vi "PicoReadPicoStreamingBuffers.vi"(1 "enabled array":i16[](array[numeric]), 2 "Buffer and Transfer Settings":T2={"startIndex"=0, "Samples"=1000000, "Down Sample Ratio"=1, "Down-Sample Mode"=2147483648} {"Down-Sample Mode" items=["RAW none"=2147483648, "None"=0, "Aggregate"=1, "Decimate"=2, "Average"=4]; "Down Sample Ratio" step=1; "Samples" format="%_6p"}, 3 "Variant":string, 5 "Pointer array":u64[][](array[numeric]), 7 "Offset Index":u32, 9 "Number of Samples":u32, 11 "error in (no error)":errorcluster) -> (6 "Buffers (Max or non-aggregated)":T1, 8 "Buffers (Min)":T1, 15 "error out":errorcluster)   [LabVIEW 2010]
doc: "Read data from Picodata buffers for streaming examples"
uses:
  Buffer and Transfer Settings.ctl
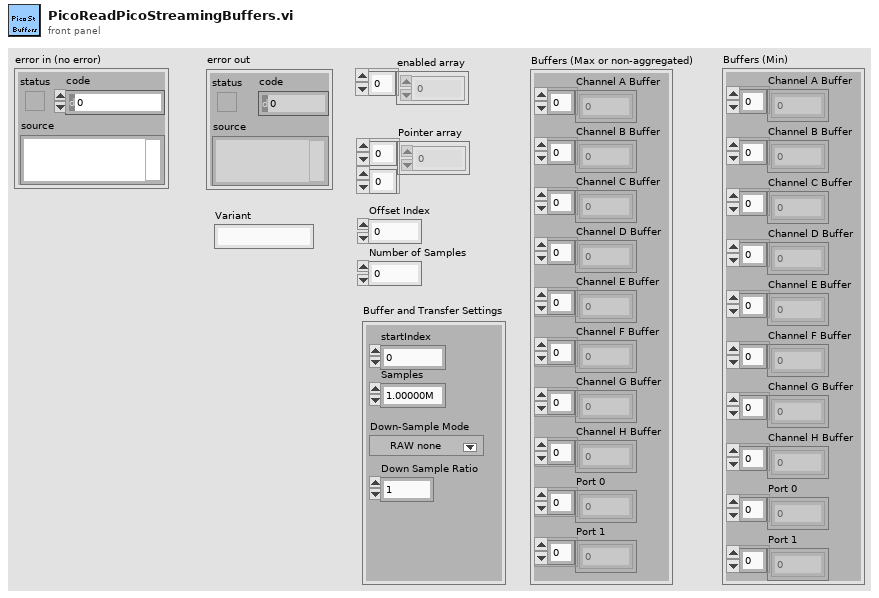
[diagram p1: front panel]
types:
  T1 = cluster{"Channel A Buffer":i16[], "Channel B Buffer":i16[], "Channel C Buffer":i16[], "Channel D Buffer":i16[], "Channel E Buffer":i16[], "Channel F Buffer":i16[], "Channel G Buffer":i16[], "Channel H Buffer":i16[], "Port 0":i16[], "Port 1":i16[]}
  T2 = typedef "Buffer and Transfer Settings.ctl" = cluster{"startIndex":u64, "Samples":u64, "Down Sample Ratio":u64, "Down-Sample Mode":u32}
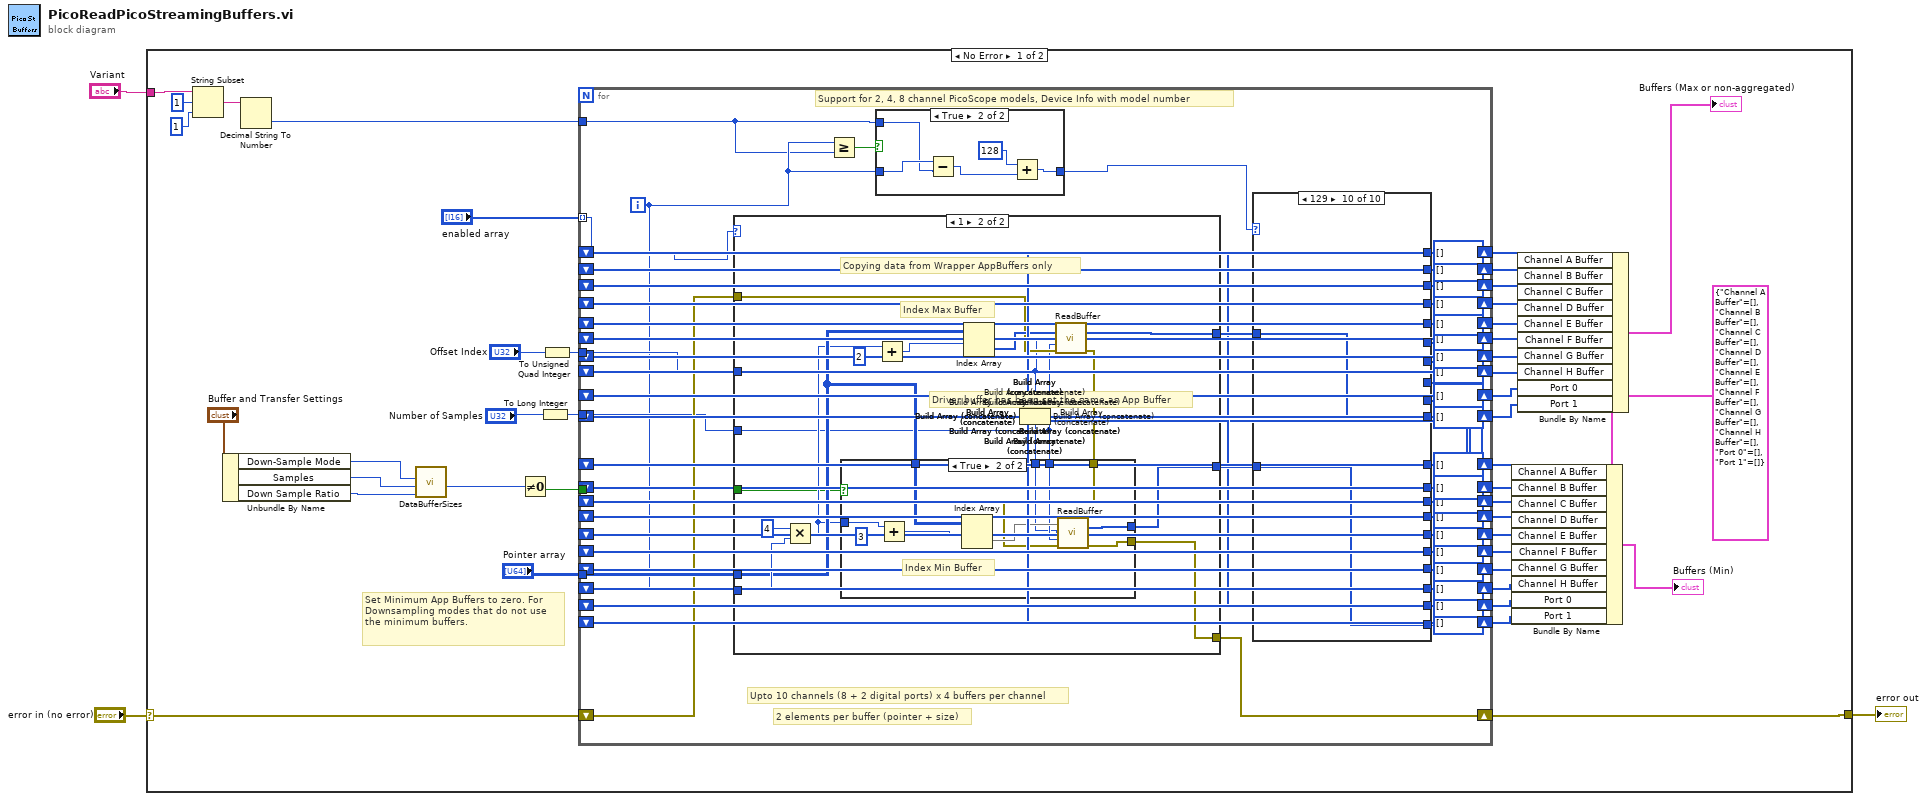
[diagram p0: block diagram]
diagram:
  n1 = case shown="No Error" "error in (no error)" {
    selector: "error in (no error)" -> [w62 w192]
    tunnel: [w64 w192] -> w2
    tunnel: "Variant" -> [w29 _]
    frame No Error {
      w39 = T1 {"Channel A Buffer"=[], "Channel B Buffer"=[], "Channel C Buffer"=[], "Channel D Buffer"=[], "Channel E Buffer"=[], "Channel F Buffer"=[], "Channel G Buffer"=[], "Channel H Buffer"=[], "Port 0"=[], "Port 1"=[]} ("Buffers (Max or non-aggregated)")
      # "Set Minimum App Buffers to zero. For Downsampling modes that do not use the minimum buffers."
      n2 = String Subset(string=w29, offset (0)=1, length (rest)=1 ("length (rest)")) -> (substring=w26:string)
      n3 = Unbundle By Name("Buffer and Transfer Settings") -> ("Down-Sample Mode"=w49:u32, "Samples"=w48:u64, "Down Sample Ratio"=w50:u64)
      n4 = Decimal String To Number(string=w26) -> (number=w24:i32)  [unwired: 2 in, 1 out]
      n5 = call "DataBufferSizes.vi"("Down Sample Ratio"=w50, "Number of Samples"=w48, "Down-Sample Mode"=w49) -> ("min Buffer Size"=w46:i32)  [unwired: 7 in, 1 out]
      n6 = Not Equal To 0?(x=w46) -> (x != 0?=w47:bool)
      n7 = To Long Integer(number="Number of Samples") -> (32bit integer=w41:i32)
      n8 = To Unsigned Quad Integer(1:"Offset Index") -> (0:w44:u64)
      n9 = for {
        tunnel: "enabled array" -> [w137] mode=indexing
        tunnel: "Pointer array" -> [w138]
        shift-right: [w136] -> w64
        shift-left: w62 -> [w135]
        tunnel: w41 -> [w121]
        tunnel: w47 -> [w120]
        tunnel: w44 -> [w118]
        tunnel: w24 -> [w106]
        shift-right: [w104] -> w61
        shift-left: i16[] [] ("Output Array") -> [w105]
        shift-right: [w102] -> w60
        shift-left: i16[] [] ("Output Array") -> [w103]
        shift-right: [w100] -> w59
        shift-left: i16[] [] ("Output Array") -> [w101]
        shift-right: [w98] -> w58
        shift-left: i16[] [] ("Output Array") -> [w99]
        shift-right: [w96] -> w57
        shift-left: i16[] [] ("Output Array") -> [w97]
        shift-right: [w94] -> w56
        shift-left: i16[] [] ("Output Array") -> [w95]
        shift-right: [w92] -> w45
        shift-left: i16[] [] ("Output Array") -> [w93]
        shift-right: [w90] -> w55
        shift-left: i16[] [] ("Output Array") -> [w91]
        shift-right: [w88] -> w54
        shift-left: i16[] [] ("Output Array") -> [w89]
        shift-right: [w86] -> w53
        shift-left: i16[] [] ("Output Array") -> [w87]
        shift-right: [w84] -> w52
        shift-left: i16[] [] ("Output Array") -> [w85]
        shift-right: [w82] -> w51
        shift-left: i16[] [] ("Output Array") -> [w83]
        shift-right: [w80] -> w36
        shift-left: i16[] [] ("Output Array") -> [w81]
        shift-right: [w78] -> w35
        shift-left: i16[] [] ("Output Array") -> [w79]
        shift-right: [w76] -> w37
        shift-left: i16[] [] ("Output Array") -> [w77]
        shift-right: [w74] -> w34
        shift-left: i16[] [] ("Output Array") -> [w75]
        shift-right: [w72] -> w33
        shift-left: i16[] [] ("Output Array") -> [w73]
        shift-right: [w70] -> w32
        shift-left: i16[] [] ("Output Array") -> [w71]
        shift-right: [w68] -> w31
        shift-left: i16[] [] ("Output Array") -> [w69]
        shift-right: [w66] -> w30
        shift-left: i16[] [] ("Output Array") -> [w67]
        i -> [w108]
        # "Support for 2, 4, 8 channel PicoScope models, Device Info with model number"
        # "2 elements per buffer (pointer + size)"
        # "Upto 10 channels (8 + 2 digital ports) x 4 buffers per channel"
        n10 = case shown="1" w137 {
          tunnel: w138 -> [_ w178]
          tunnel: w108 -> [_ w179]
          tunnel: [_ w173] -> w134
          tunnel: [_ w172] -> w133
          tunnel: w135 -> [w165 w171]
          tunnel: [w165 w169] -> w136
          tunnel: w121 -> [_ w167]
          tunnel: w120 -> [_ w168]
          tunnel: w118 -> [_ w166]
          frame 0, Default {
          }
          frame 1 {
            # "Driver buffer has been set the same as App Buffer"
            # "Copying data from Wrapper AppBuffers only"
            # "Index Max Buffer"
            n11 = Multiply(x=4, y=w179) -> (x*y=w175:i32)
            n12 = Add(x=w175, y=2) -> (x+y=w177:i32)
            n13 = Index Array(array=w178, index (row)=w177) -> (element=w174:u64[])  [unwired: 1 in]
            n14 = call "ReadBuffer.vi"("Pointer and BufferSize"=w174, "Offset"=w166, "Buffer size"=w167, "error in (no error)"=w171) -> ("Output Array"=w173:i16[], "error out"=w170:errorcluster)  [unwired: 10 in]
            n15 = case shown="True" w168 {
              tunnel: w178 -> [_ w191]
              tunnel: w175 -> [_ w188]
              tunnel: [_ w186] -> w172
              tunnel: w170 -> [w181 w185]
              tunnel: [w181 w184] -> w169
              tunnel: w167 -> [_ w183]
              tunnel: w166 -> [_ w182]
              frame False {
              }
              frame True {
                # "Index Min Buffer"
                n16 = Add(x=w188, y=3) -> (x+y=w189:i32)
                n17 = Index Array(array=w191, index (row)=w189) -> (element=w187:u64[])  [unwired: 1 in]
                n18 = call "ReadBuffer.vi"("Pointer and BufferSize"=w187, "Offset"=w182, "Buffer size"=w183, "error in (no error)"=w185) -> ("Output Array"=w186:i16[], "error out"=w184:errorcluster)  [unwired: 10 in]
              }
            }
          }
        }
        n19 = Greater Or Equal?(x=w108, y=w106) -> (x >= y?=w109:bool)
        n20 = case shown="True" w109 {
          tunnel: w108 -> [w139 w141]
          tunnel: [w139 w143] -> w107
          tunnel: w106 -> [_ w140]
          frame False {
          }
          frame True {
            n21 = Subtract(x=w141, y=w140) -> (x-y=w142:i32)
            n22 = Add(x=128, y=w142) -> (x+y=w143:i32)
          }
        }
        n23 = case shown="129" w107 {
          tunnel: w134 -> [w146 w148 w150 w152 w154 w156 w158 w160 w162 w163]
          tunnel: [w146 _ _ _ _ _ _ _ _ _] -> w119
          tunnel: [_ w148 _ _ _ _ _ _ _ _] -> w126
          tunnel: [_ _ w150 _ _ _ _ _ _ _] -> w125
          tunnel: [_ _ _ w152 _ _ _ _ _ _] -> w124
          tunnel: [_ _ _ _ w154 _ _ _ _ _] -> w123
          tunnel: [_ _ _ _ _ w156 _ _ _ _] -> w122
          tunnel: w133 -> [w145 w147 w149 w151 w153 w155 w157 w159 w161 w164]
          tunnel: [w145 _ _ _ _ _ _ _ _ _] -> w132
          tunnel: [_ w147 _ _ _ _ _ _ _ _] -> w131
          tunnel: [_ _ w149 _ _ _ _ _ _ _] -> w130
          tunnel: [_ _ _ w151 _ _ _ _ _ _] -> w129
          tunnel: [_ _ _ _ w153 _ _ _ _ _] -> w128
          tunnel: [_ _ _ _ _ w155 _ _ _ _] -> w127
          tunnel: [_ _ _ _ _ _ w158 _ _ _] -> w117
          tunnel: [_ _ _ _ _ _ _ w160 _ _] -> w116
          tunnel: [_ _ _ _ _ _ w157 _ _ _] -> w115
          tunnel: [_ _ _ _ _ _ _ w159 _ _] -> w114
          tunnel: [_ _ _ _ _ _ _ _ w162 _] -> w113
          tunnel: [_ _ _ _ _ _ _ _ w161 _] -> w112
          tunnel: [_ _ _ _ _ _ _ _ _ w164] -> w111
          tunnel: [_ _ _ _ _ _ _ _ _ w163] -> w110
          frame 0, Default {
          }
          frame 1 {
          }
          frame 2 {
          }
          frame 3 {
          }
          frame 4 {
          }
          frame 5 {
          }
          frame 6 {
          }
          frame 7 {
          }
          frame 128 {
          }
          frame 129 {
          }
        }
        n24 = Build Array (concatenate)(w67, w110) -> (w66:i16[])
        n25 = Build Array (concatenate)(w69, w111) -> (w68:i16[])
        n26 = Build Array (concatenate)(w71, w112) -> (w70:i16[])
        n27 = Build Array (concatenate)(w73, w113) -> (w72:i16[])
        n28 = Build Array (concatenate)(w75, w114) -> (w74:i16[])
        n29 = Build Array (concatenate)(w77, w115) -> (w76:i16[])
        n30 = Build Array (concatenate)(w79, w116) -> (w78:i16[])
        n31 = Build Array (concatenate)(w81, w117) -> (w80:i16[])
        n32 = Build Array (concatenate)(w83, w122) -> (w82:i16[])
        n33 = Build Array (concatenate)(w85, w123) -> (w84:i16[])
        n34 = Build Array (concatenate)(w87, w124) -> (w86:i16[])
        n35 = Build Array (concatenate)(w89, w125) -> (w88:i16[])
        n36 = Build Array (concatenate)(w91, w126) -> (w90:i16[])
        n37 = Build Array (concatenate)(w93, w119) -> (w92:i16[])
        n38 = Build Array (concatenate)(w95, w127) -> (w94:i16[])
        n39 = Build Array (concatenate)(w97, w128) -> (w96:i16[])
        n40 = Build Array (concatenate)(w99, w129) -> (w98:i16[])
        n41 = Build Array (concatenate)(w101, w130) -> (w100:i16[])
        n42 = Build Array (concatenate)(w103, w131) -> (w102:i16[])
        n43 = Build Array (concatenate)(w105, w132) -> (w104:i16[])
      }
      n44 = Bundle By Name(cluster=w39, "Channel A Buffer"=w61, "Channel B Buffer"=w60, "Channel C Buffer"=w59, "Channel D Buffer"=w58, "Channel E Buffer"=w57, "Channel F Buffer"=w56, "Channel G Buffer"=w37, "Channel H Buffer"=w34, "Port 0"=w32, "Port 1"=w31) -> (→"Buffers (Min)":T1)
      n45 = Bundle By Name(cluster=w39, "Channel A Buffer"=w45, "Channel B Buffer"=w55, "Channel C Buffer"=w54, "Channel D Buffer"=w53, "Channel E Buffer"=w52, "Channel F Buffer"=w51, "Channel G Buffer"=w36, "Channel H Buffer"=w35, "Port 0"=w33, "Port 1"=w30) -> (→"Buffers (Max or non-aggregated)":T1)
    }
    frame Error {
    }
  }
  "error out" <- w2
